vi "LHF.DB.Mongo.Collection.Aggregate.vi"(6 "Extract _id (T)":bool=TRUE, 7 "return type":variant, 8 "error in (no error)":errorcluster, 9 "Operations":variant[](array[variant]), 10 "Collection":string, 11 "LHF.DB.Mongo in":refnum<class "LHF.DB.Mongo.lvclass">) -> (0 "error out":errorcluster, 1 "_id Array":string[](array[string]), 2 "Documents":variant[](array[variant]), 3 "LHF.DB.Mongo out":refnum<class "LHF.DB.Mongo.lvclass">)   [LabVIEW 2013, in "LHF.DB.Mongo.lvclass"]
doc: "return type: wire cluster of expected document output, then variant to data with documents output. use cluster element's name to choose what document field you're expecting\noperations: wire array of cluster variant, name the cluster variant with the desired aggregation operation as $project or $match then use element names to setup pipeline."
uses:
  LHF.DB.Mongo.lvclass
  C:/Users/Ricardo/Desktop/Projetos/LabVIEW-MongoDB/src/Driver/MongoDB.Bson.dll
  Driver/MongoDB.Bson.dll
  <userlib>/_OpenG.lib/string/string.llb/Trim Whitespace (String)__ogtk.vi
  <vilib>/Utility/VariantDataType/VariantType.lvlib
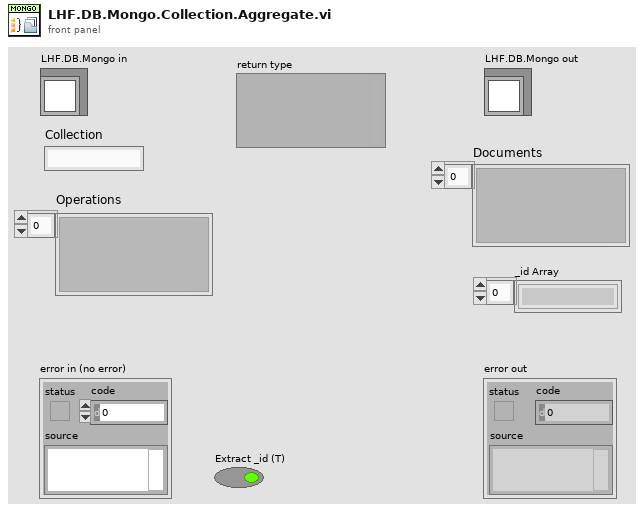
[diagram p1: front panel]
types:
  T1 = enum16{"$project", "$limit", "$skip", "$match", "$redact", "$unwind", "$group", "$sort", "$sample", "$geonear", "$lookup", "$out", "$indexstats"}
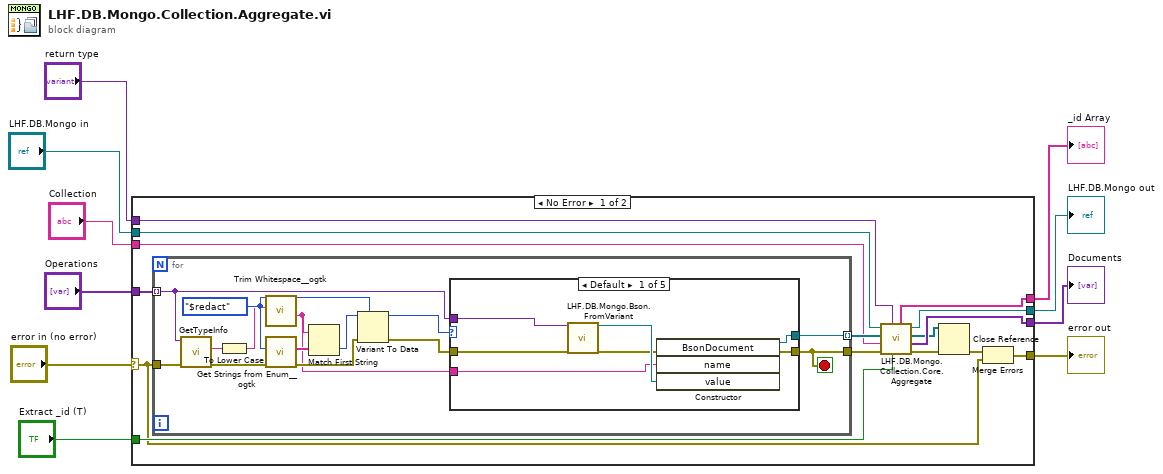
[diagram p0: block diagram]
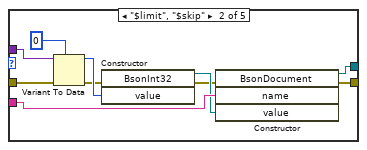
[diagram p2: hidden frame]
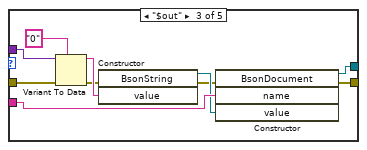
[diagram p3: hidden frame]
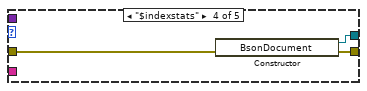
[diagram p4: hidden frame]
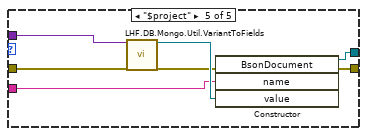
[diagram p5: hidden frame]
diagram:
  n1 = case shown="No Error" "error in (no error)" {
    selector: "error in (no error)" -> [w12 w78]
    tunnel: [w20 w78] -> w9
    tunnel: [w23 w77] -> w7
    tunnel: "LHF.DB.Mongo in" -> [w24 w77]
    tunnel: "Collection" -> [w19 _]
    tunnel: "Operations" -> [w25 _]
    tunnel: [w18 _] -> w4
    tunnel: "Extract _id (T)" -> [w17 _]
    tunnel: [w16 _] -> w2
    tunnel: "return type" -> [w11 _]
    frame No Error {
      n2 = for {
        tunnel: w25 -> [w37] mode=indexing
        tunnel: [w39] -> w21 mode=indexing
        tunnel: [w38] -> w22
        tunnel: w12 -> [w31]
        stop <- w38 stop-if-true
        w36 = T1."$redact"
        n3 = call <vilib>:"GetTypeInfo.vi"("error in (no error)"=w31, "Variant"=w37) -> ("error out"=w32:errorcluster, "Name"=w34:string)  [unwired: 5 in, 3 out]
        n4 = To Lower Case(string=w34) -> (all lower case string=w27:string)
        n5 = call-poly <userlib>:"Trim Whitespace__ogtk.vi"("String in"=w27) -> ("String out"=w26:string)  [unwired: 6 in]
        n6 = call <userlib>:"Get Strings from Enum__ogtk.vi"("error in (no error)"=w32, "Enum"=w36) -> ("error out"=w33:errorcluster, "Enum Strings"=w29:string[])  [unwired: 6 in, 2 out]
        n7 = Match First String(2:w29, 3:w26) -> (0:w35:i32)  [unwired: 1 out]
        n8 = Variant To Data(error in=w33, type=w36, Variant=w35) -> (data=w28:T1, error out=w30:errorcluster)
        n9 = case shown="Default" w28 {
          tunnel: [w42 w52 w62 w69 w72] -> w39
          tunnel: [w41 w47 w57 w68 w71] -> w38
          tunnel: w30 -> [w45 w54 w64 w67 w76]
          tunnel: w37 -> [w46 w56 w66 _ w75]
          tunnel: w26 -> [w40 w53 w63 _ w70]
          frame Default {
            n10 = call "LHF.DB.Mongo.Bson.FromVariant.vi"("Variant"=w46, "error IO"=w45) -> ("BsonValue"=w44:refnum<k24>, "error IO 2"=w43:errorcluster)  [unwired: 16 in]
            n11 = constructor class="BsonDocument"(error in=w43, "name"=w40, "value"=w44) -> (reference out=w42:refnum<k24>, error out=w41:errorcluster)  [unwired: 2 in, 3 out]
          }
          frame "$limit", "$skip" {
            n12 = Variant To Data(error in=w54, type=0, Variant=w56) -> (data=w51:i32, error out=w50:errorcluster)
            n13 = constructor class="BsonInt32"(error in=w50, "value"=w51) -> (reference out=w49:refnum<k24>, error out=w48:errorcluster)  [unwired: 2 in, 2 out]
            n14 = constructor class="BsonDocument"(error in=w48, "name"=w53, "value"=w49) -> (reference out=w52:refnum<k24>, error out=w47:errorcluster)  [unwired: 2 in, 3 out]
          }
          frame "$out" {
            n15 = Variant To Data(error in=w64, type="0", Variant=w66) -> (data=w61:string, error out=w60:errorcluster)
            n16 = constructor class="BsonString"(error in=w60, "value"=w61) -> (reference out=w59:refnum<k24>, error out=w58:errorcluster)  [unwired: 2 in, 2 out]
            n17 = constructor class="BsonDocument"(error in=w58, "name"=w63, "value"=w59) -> (reference out=w62:refnum<k24>, error out=w57:errorcluster)  [unwired: 2 in, 3 out]
          }
          frame "$indexstats" {
            n18 = constructor class="BsonDocument"(error in=w67) -> (reference out=w69:refnum<k24>, error out=w68:errorcluster)  [unwired: 2 in, 1 out]
          }
          frame "$project" {
            n19 = call "LHF.DB.Mongo.Util.VariantToFields.vi"("projection type"=w75, "error in (no error)"=w76) -> ("BsonDocument"=w74:refnum<k24>, "error out"=w73:errorcluster)  [unwired: 16 in]
            n20 = constructor class="BsonDocument"(error in=w73, "name"=w70, "value"=w74) -> (reference out=w72:refnum<k24>, error out=w71:errorcluster)  [unwired: 2 in, 3 out]
          }
        }
      }
      n21 = call "LHF.DB.Mongo.Collection.Core.Aggregate.vi"("Extract _id"=w17, "type"=w11, "error in (no error)"=w22, "Collection"=w19, "operations"=w21, "LHF.DB.Mongo in"=w24) -> ("error out"=w14:errorcluster, "Documents"=w18:variant[], "operations out"=w15:refnum<k24>[], "LHF.DB.Mongo out"=w23:refnum<class "LHF.DB.Mongo.lvclass">, "_id Array"=w16:string[])  [unwired: 1 in]
      n22 = Close Reference(reference=w15, error in (no error)=w14) -> (error out=w13:errorcluster)
      n23 = Merge Errors(w13, w12) -> (w20:errorcluster)
    }
    frame Error {
    }
  }
  "error out" <- w9
  "LHF.DB.Mongo out" <- w7
  "Documents" <- w4
  "_id Array" <- w2
